vi "CO stop TurnTable.vi"(8 "error in (no error)":errorcluster caption="에러 입력(에러 없음)", 11 "Instrument Manager 입력":refnum<class "Instrument Manager.lvclass">) -> (0 "error out":errorcluster caption="에러 출력", 3 "Instrument Manager 출력":refnum<class "Instrument Manager.lvclass">)   [LabVIEW 2023, in "Instrument Manager.lvclass"]
uses:
  Instrument Manager.lvclass
  Instrument Manager.lvclass/Instrument Manager.ctl
  Module/Turn Table and Mast Control/Interface Class/Turn Table/Interface - Turn Table.lvclass
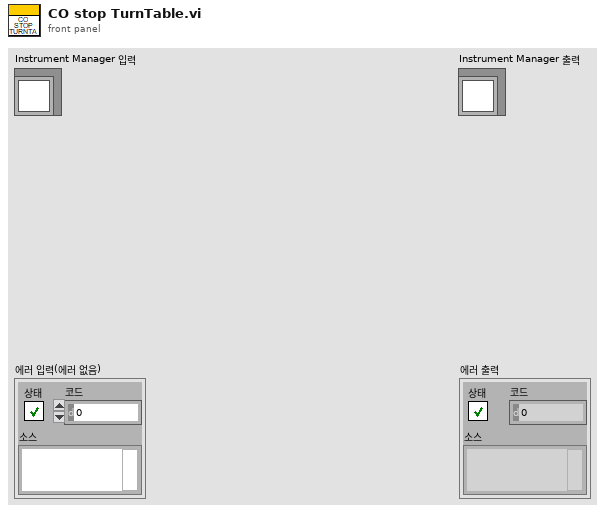
[diagram p1: front panel]
types:
  T1 = cluster{"Anritsu Call Box":refnum<class "Anritsu Call Box.lvclass">, "Spectrum Analyzer":refnum<class "Interface_Spectrum.lvclass">, "RF Switch Box":refnum<class "RF Filter Box.lvclass">, "Turn Table":refnum<class "Interface - Turn Table.lvclass">, "Mast":refnum<class "Interface - Mast.lvclass">, "3D Controller":refnum<class "Interface_3D Controller.lvclass">}
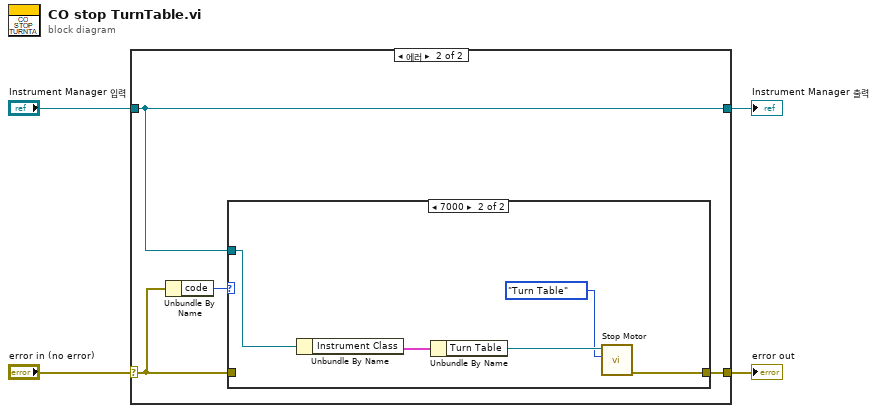
[diagram p0: block diagram]
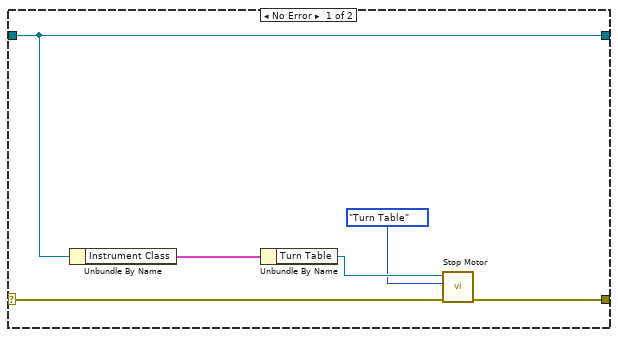
[diagram p2: hidden frame]
diagram:
  n1 = case shown="에러" "error in (no error)" {
    selector: "error in (no error)" -> [w8 w13]
    tunnel: [w7 w12] -> w3
    tunnel: [w10 w11] -> w1
    tunnel: "Instrument Manager 입력" -> [w10 w11]
    frame No Error {
      n2 = Unbundle By Name(w10) -> ("Instrument Class"=w9:T1)
      n3 = Unbundle By Name(w9) -> ("Turn Table"=w6:refnum<class "Interface - Turn Table.lvclass">)
      n4 = call-dynamic "Stop Motor.vi"("error in (no error)"=w8, "Target"=enum16{"Mast", "Turn Table"}."Turn Table", "Interface - Turn Table in"=w6) -> ("error out"=w7:errorcluster)  [unwired: 7 in, 1 out]
    }
    frame Error {
      n5 = Unbundle By Name(w13) -> ("code"=w14:i32)
      n6 = case shown="7000" w14 {
        tunnel: w13 -> [w15 _]
        tunnel: [w15 w17] -> w12
        tunnel: w11 -> [_ w16]
        frame 0, Default {
        }
        frame 7000 {
          n7 = Unbundle By Name(w16) -> ("Instrument Class"=w20:T1)
          n8 = Unbundle By Name(w20) -> ("Turn Table"=w19:refnum<class "Interface - Turn Table.lvclass">)
          n9 = call-dynamic "Stop Motor.vi"("Target"=enum16{"Mast", "Turn Table"}."Turn Table", "Interface - Turn Table in"=w19) -> ("error out"=w17:errorcluster)  [unwired: 8 in, 1 out]
        }
      }
    }
  }
  "error out" <- w3
  "Instrument Manager 출력" <- w1
